vi "Generer_listing_alarmes.vi"(1 "Configuration":cluster{"Command (PV)":string, dbl}[](array[cluster]) {"?" format="%#.1f"}) -> (0 "Listing alarmes":string)   [LabVIEW 2022 SP3]
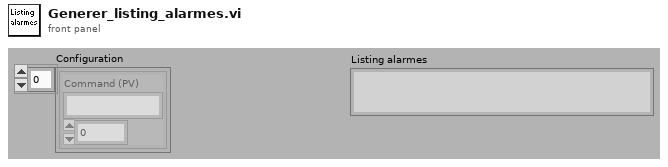
[diagram p1: front panel]
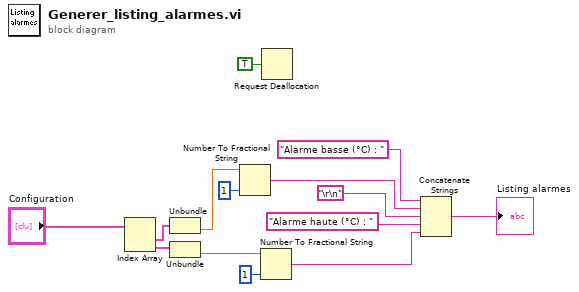
[diagram p0: block diagram]
diagram:
  n1 = Index Array(array="Configuration") -> (element #1=w11:cluster{"Command (PV)":string, dbl}, element #2=w10:cluster{"Command (PV)":string, dbl})  [unwired: 2 in]
  n2 = Unbundle(w11) -> (w6:dbl)  [unwired: 1 out]
  n3 = Unbundle(w10) -> (w4:dbl)  [unwired: 1 out]
  n4 = Number To Fractional String(number=w6, precision (6)=i16 1 ("précision (6)")) -> (F-format string=w5:string)  [unwired: 2 in]
  n5 = Number To Fractional String(number=w4, precision (6)=i16 1 ("précision (6)")) -> (F-format string=w3:string)  [unwired: 2 in]
  n6 = Request Deallocation(TRUE ("flag")) -> ()
  n7 = Concatenate Strings("Alarme basse (°C) : " ("chaîne"), w5, "\r\n", "Alarme haute (°C) : " ("chaîne"), w3) -> (→"Listing alarmes":string)
